vi "Read Object Property.vi"(8 "error in":errorcluster, 10 "property name":string, 11 "object in":T1) -> (0 "error out":errorcluster, 2 "value":T1, 3 "object out":T1)   [LabVIEW 2026, in "ToastNotification.lvlib" / "Reflection DotNet.lvlib"]
doc: "Read a named public property of a borrowed .NET object through reflection. Release acquired Type and PropertyInfo metadata on success and failure. value is an acquired boxed property value and must be closed by its caller, including on error. object out is the same borrowed input alias, preserved even on incoming error; never close it as a second acquisition. Skip property acquisition on incoming error."
uses:
  Reflection DotNet.lvlib
  Callback Object Reference.ctl
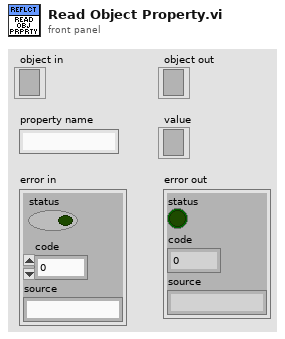
[diagram p1: front panel]
types:
  T1 = typedef "ToastNotification.lvlib/Reflection DotNet.lvlib/Callback Object Reference.ctl" = refnum<k24>
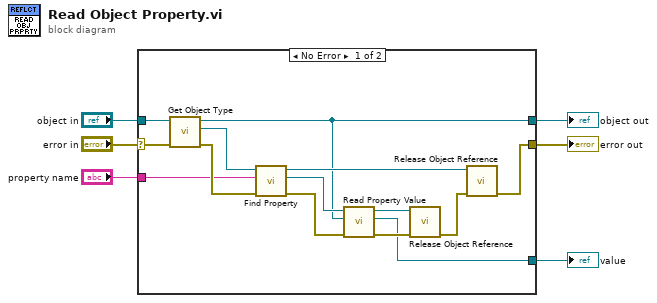
[diagram p0: block diagram]
diagram:
  n1 = case shown="No Error" "error in" {
    selector: "error in" -> [w13 w22]
    tunnel: "object in" -> [w8 w21]
    tunnel: "property name" -> [w14 _]
    tunnel: [w17 _] -> w5
    tunnel: [w20 w22] -> w6
    tunnel: [w7 w21] -> w1
    frame No Error {
      n2 = call "Get Object Type.vi"("error in (no error)"=w13, "Object in"=w8) -> ("error out"=w15:errorcluster, "Object Type"=w10:refnum<k24>, "Object out"=w7:refnum<k24>)  [unwired: 7 in]
      n3 = call "Find Property.vi"("error in (no error)"=w15, "Property Name"=w14, "Object Type in"=w10) -> ("error out"=w16:errorcluster, "Property Info"=w12:refnum<k24>, "Object Type out"=w9:refnum<k24>)  [unwired: 6 in]
      n4 = call "Read Property Value.vi"("error in (no error)"=w16, "Target Object"=w7, "Property Info in"=w12) -> ("error out"=w18:errorcluster, "Property Value"=w17:refnum<k24>, "Property Info out"=w11:refnum<k24>)  [unwired: 6 in]
      n5 = call "Release Object Reference.vi"("error in"=w18, "object"=w11) -> ("error out"=w19:errorcluster)  [unwired: 9 in]
      n6 = call "Release Object Reference.vi"("error in"=w19, "object"=w9) -> ("error out"=w20:errorcluster)  [unwired: 9 in]
    }
    frame Error {
    }
  }
  "value" <- w5
  "error out" <- w6
  "object out" <- w1
